vi "generate table.vi"(5 "assemblies":refnum<vi>, 7 "table":refnum<vi>, 8 "error in":errorcluster, 10 "engine configuration in":refnum<class "engine configuration.lvclass">, 11 "EthernetIP configuration in":refnum<class "EIP Tags Configuration.lvclass">) -> (0 "error out":errorcluster)   [LabVIEW 2013, in "EIP Tags editor node.lvclass"]
uses:
  EIP Tags editor node.lvclass
  table line.ctl
  <vilib>/NI/Module Execution Interface/Engine Configuration/engine configuration.lvclass
  <vilib>/NI/Tag Bus/tag/tag descriptor.lvclass
  configuration/EIP Tags Configuration.lvclass
  channel/EIP Tags Channel.lvclass
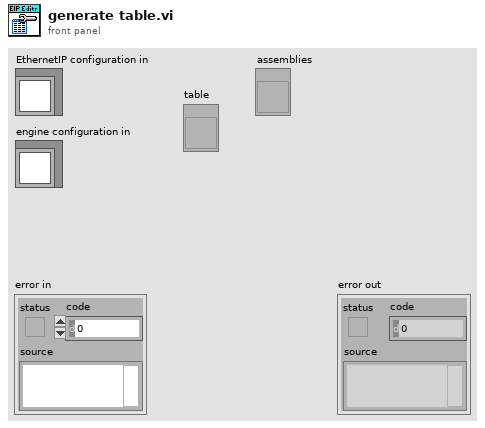
[diagram p1: front panel]
types:
  T1 = typedef "EIP Tags Configuration.lvclass/eip tag definition.ctl" = cluster{"eip tag types":T2, "unique tag name":string, "Number of Elements":u32}
  T2 = typedef "EIP Tags Configuration.lvclass/eip tag types.ctl" = enum16{"SINT", "INT", "DINT", "REAL", "BOOL", "STRING"}
  T3 = typedef "EIP Tags editor node.lvclass/table line.ctl" = cluster{"eip channel":refnum<class "EIP Tags Channel.lvclass">, "tag name":string}
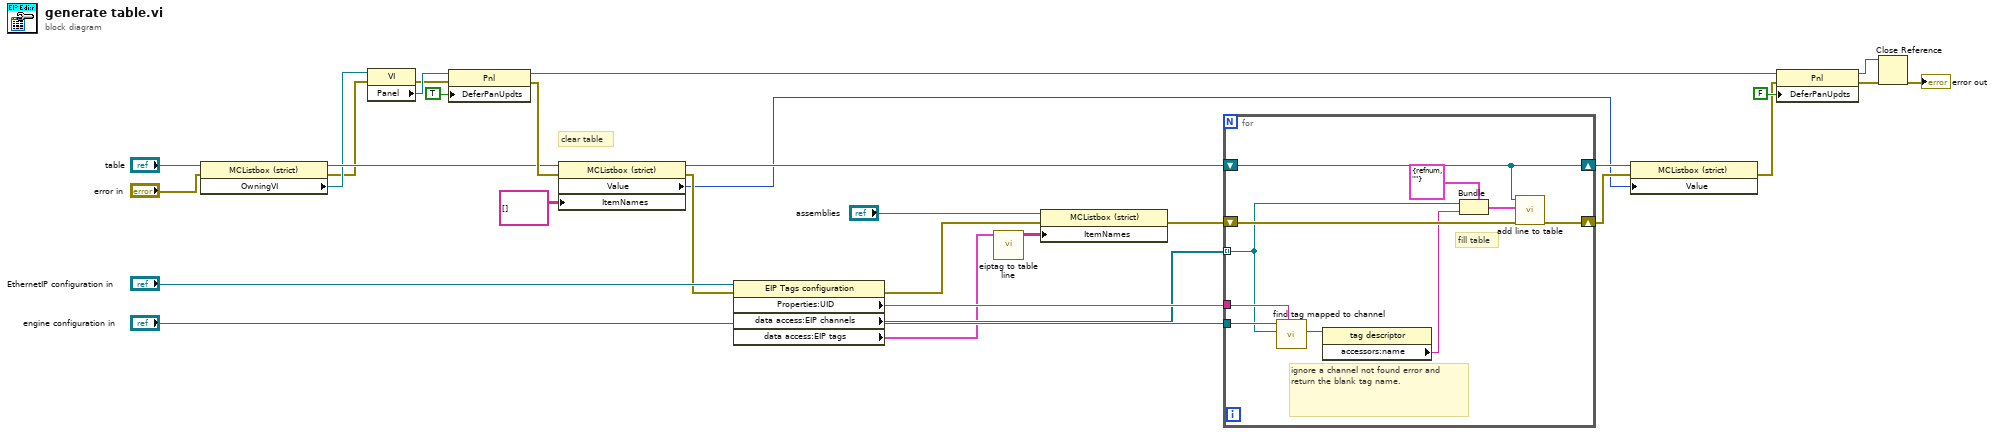
[diagram p0: block diagram]
diagram:
  # "clear table"
  n1 = property class="MCListbox (strict)"(reference="table", error in="error in") -> (reference out=w12:refnum<vi>, error out=w9:errorcluster, "OwningVI"=w10:refnum<vi>)
  n2 = property class="VI"(reference=w10, error in=w9) -> (error out=w18:errorcluster, "Panel"=w19:refnum<vi>)  [unwired: 1 out]
  n3 = property class="Pnl"(reference=w19, error in=w18, "DeferPanUpdts"=TRUE ("Defer Panel Updates")) -> (reference out=w15:refnum<vi>, error out=w17:errorcluster)
  n4 = property class="MCListbox (strict)"(reference=w12, error in=w17, "ItemNames"=string[][] [] ("Item Names")) -> (reference out=w29:refnum<vi>, error out=w25:errorcluster, "Value"=w21:i32)
  n5 = property class="EIP Tags configuration"(reference="EthernetIP configuration in", error in=w25) -> (error out=w4:errorcluster, "Properties:UID"=w26:string, "data access:EIP channels"=w6:refnum<class "EIP Tags Channel.lvclass">[], "data access:EIP tags"=w5:T1[])  [unwired: 1 out]
  n6 = call "eiptag to table line.vi"("eip tags"=w5) -> ("Item Names"=w1:string[][])  [unwired: 10 in]
  n7 = property class="MCListbox (strict)"(reference="assemblies", error in=w4, "ItemNames"=w1) -> (error out=w3:errorcluster)  [unwired: 1 out]
  n8 = for {
    shift-right: [w40] -> w22
    shift-left: w3 -> [w37]
    tunnel: w6 -> [w34] mode=indexing
    tunnel: "engine configuration in" -> [w36]
    tunnel: w26 -> [w35]
    shift-right: [w31] -> w23
    shift-left: w29 -> [w31]
    # "ignore a channel not found error and return the blank tag name."
    # "fill table"
    n9 = call <vilib>:"find tag mapped to channel.vi"("owner"=w35, "channel"=w34, "engine configuration in"=w36) -> ("tag"=w33:refnum<class "tag descriptor.lvclass">)  [unwired: 6 in, 2 out]
    n10 = property class="tag descriptor"(reference=w33) -> ("accessors:name"=w32:string)  [unwired: 1 in, 2 out]
    n11 = Bundle(cluster=T3 {"eip channel"=refnum, "tag name"=""} ("line"), "eip channel"=w34, "tag name"=w32) -> (w38:T3)
    n12 = call "add line to table.vi"("error in"=w37, "line"=w38, "operations table"=w31) -> ("error out"=w40:errorcluster)  [unwired: 8 in]
  }
  n13 = property class="MCListbox (strict)"(reference=w23, error in=w22, "Value"=w21) -> (error out=w14:errorcluster)  [unwired: 1 out]
  n14 = property class="Pnl"(reference=w15, error in=w14, "DeferPanUpdts"=FALSE ("Defer Panel Updates")) -> (reference out=w7:refnum<vi>, error out=w13:errorcluster)
  n15 = Close Reference(reference=w7, error in (no error)=w13) -> (error out=→"error out":errorcluster)
